vi "GT_StepText.vi"(11 "Step":u16) -> (3 "Step Text":string)   [LabVIEW 2026]
doc: "Use this template to build a VI to use as a subVI."
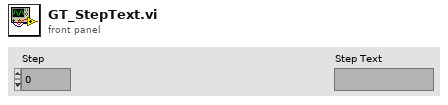
[diagram p1: front panel]
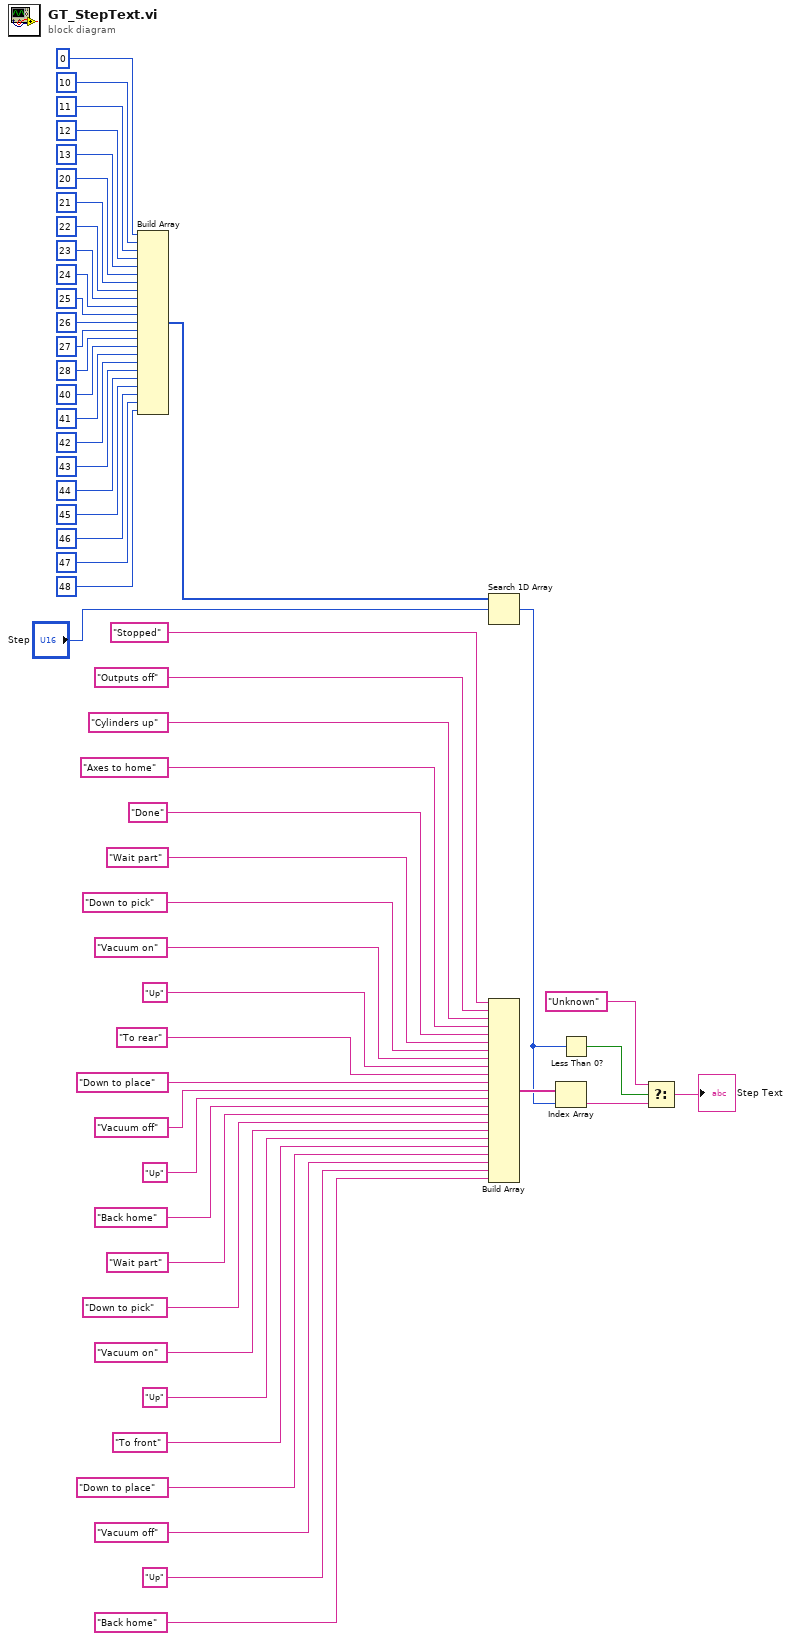
[diagram p0: block diagram]
diagram:
  n1 = Build Array(0, 10, 11, 12, 13, 20, 21, 22, 23, 24, 25, 26, 27, 28, 40, 41, 42, 43, 44, 45, 46, 47, 48) -> (w8:i32[])
  n2 = Search 1D Array(1D array=w8, element="Step") -> (index of element=w5:i32)  [unwired: 1 in]
  n3 = Build Array("Stopped", "Outputs off", "Cylinders up", "Axes to home", "Done", "Wait part", "Down to pick", "Vacuum on", "Up", "To rear", "Down to place", "Vacuum off", "Up", "Back home", "Wait part", "Down to pick", "Vacuum on", "Up", "To front", "Down to place", "Vacuum off", "Up", "Back home") -> (w6:string[])
  n4 = Index Array(array=w6, index=w5) -> (element=w2:string)
  n5 = Less Than 0?(x=w5) -> (x < 0?=w4:bool)
  n6 = Select(t="Unknown", s=w4, f=w2) -> (s? t:f=→"Step Text":string)
